vi "Host_main_Lab7.vi"() -> ()   [LabVIEW 2025]
uses:
  vi/thresholds.ctl
  RT_Cmd.ctl
  Command.ctl
  UI_Msg.ctl
  action.ctl
panel:
  out "error out":errorcluster
  in  "Manual trigger":bool
  in  "parameters":T1
  out "Waveform Graph":i16[][](graph)
  in  "Stop":bool
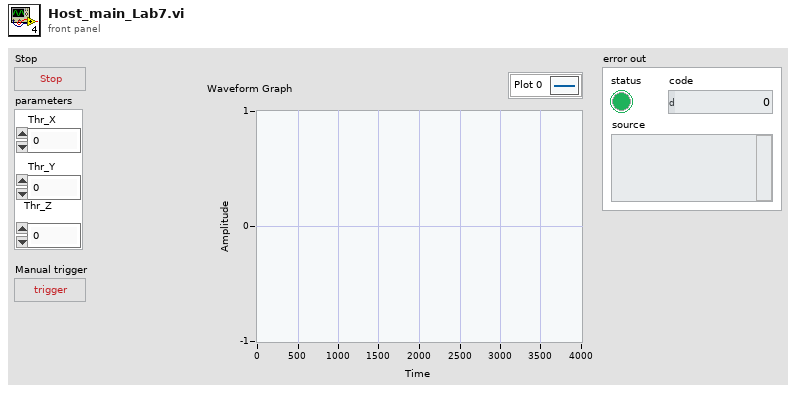
[diagram p1: front panel]
types:
  T1 = typedef "thresholds.ctl" = cluster{"Thr_X":i16, "Thr_Y":i16, "Thr_Z":i16}
  T2 = typedef "UI_Msg.ctl" = cluster{"action":T3, "Threshold":T1}
  T3 = typedef "action.ctl" = enum16{"Thresholds_Changed", "Manual_Trigger", "Stop"}
  T4 = typedef "RT_Cmd.ctl" = cluster{"command":T5, "parameters":T1}
  T5 = typedef "Command.ctl" = enum16{"threshold_config", "manual_trigger", "stop"}
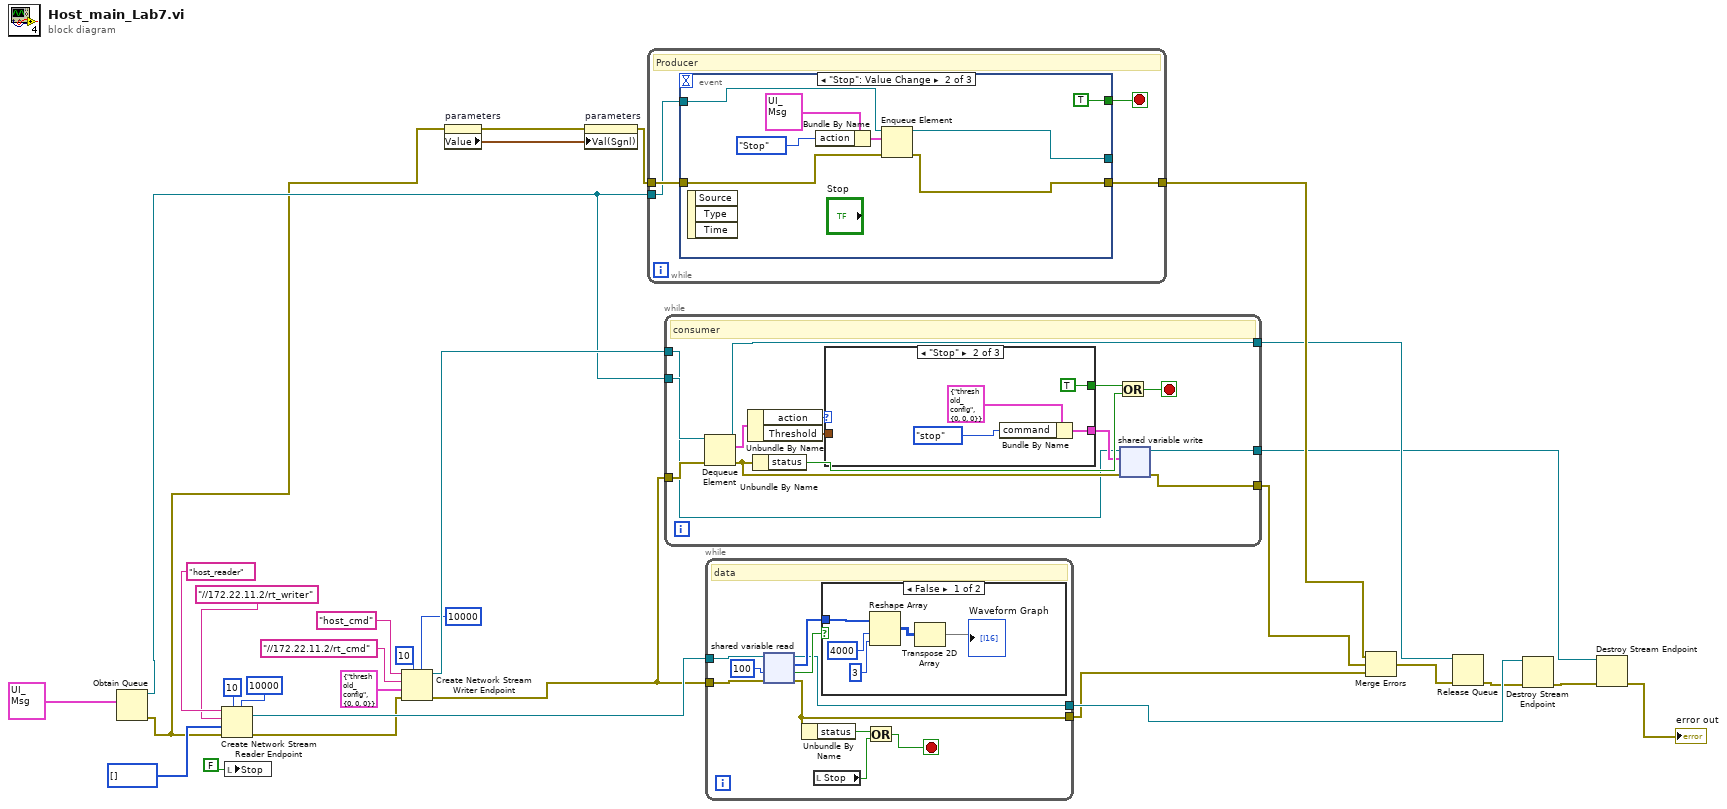
[diagram p0: block diagram]
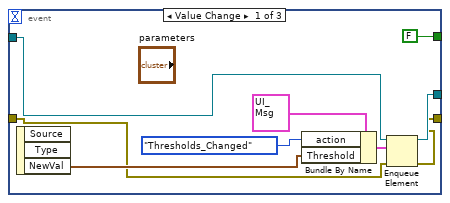
[diagram p2: hidden frame]
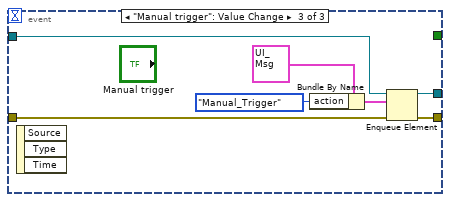
[diagram p3: hidden frame]
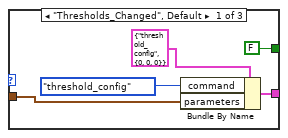
[diagram p4: hidden frame]
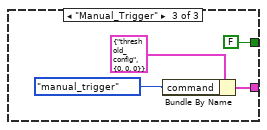
[diagram p5: hidden frame]
diagram:
  n1 = Obtain Queue(element data type=T2 {"action"=enum."Thresholds_Changed", "Threshold"={"Thr_X"=0, "Thr_Y"=0, "Thr_Z"=0}} ("msg")) -> (queue out=w5:refnum<queue>, error out=w2:errorcluster)  [unwired: 4 in, 1 out]
  n2 = Create Network Stream Reader Endpoint(5:10000 ("timeout in ms (-1)"), 7:10 ("reader buffer size"), 8:w2, 9:i16[] [], 10:"//172.22.11.2/rt_writer" ("writer url"), 11:"host_reader" ("writer name")) -> (0:w11:errorcluster, 3:w27:refnum<k21>)  [unwired: 1 in]
  n3 = local write "Stop"(FALSE ("Stop")) -> ()
  n4 = Create Network Stream Writer Endpoint(5:10000 ("timeout in ms (-1)"), 7:10 ("writer buffer size"), 8:w11, 9:T4 {"command"=enum."threshold_config", "parameters"={"Thr_X"=0, "Thr_Y"=0, "Thr_Z"=0}} ("data"), 10:"//172.22.11.2/rt_cmd" ("writer url"), 11:"host_cmd" ("writer name")) -> (0:w9:errorcluster, 3:w20:refnum<k21>)  [unwired: 1 in]
  n5 = property on="parameters" class="Clust (strict)"(error in=w2) -> (error out=w4:errorcluster, "Value"=w3:T1)  [unwired: 1 in, 1 out]
  n6 = property on="parameters" class="Clust (strict)"(error in=w4, "Val(Sgnl)"=w3) -> (error out=w1:errorcluster)  [unwired: 1 in, 1 out]
  n7 = while {
    tunnel: w1 -> [w34]
    tunnel: w5 -> [w32]
    tunnel: [w33] -> w17
    stop <- w35 stop-if-true
    # "Producer"
    n8 = event shown="[1] \"Stop\": Value Change" {
      selector: _ -> [_ _ _]
      dyn-events: _ -> [_ _ _]
      timeout: _ -> [_ _ _]
      tunnel: [FALSE TRUE _] -> w35
      tunnel: [w39 w48 w57] -> _
      tunnel: w34 -> [w38 w47 w56]
      tunnel: [w37 w46 w55] -> w33
      tunnel: w32 -> [w40 w49 w54]
      event Value Change {
        n9 = event-data() -> ("NewVal"=w41:T1)  [unwired: 1 in, 2 out]
        n10 = Bundle By Name(cluster=T2 {"action"=enum."Thresholds_Changed", "Threshold"={"Thr_X"=0, "Thr_Y"=0, "Thr_Z"=0}} ("msg"), "action"=action."Thresholds_Changed", "Threshold"=w41) -> (w43:T2)
        n11 = Enqueue Element(queue=w40, element=w43, error in (no error)=w38) -> (queue out=w39:refnum<queue>, error out=w37:errorcluster)  [unwired: 1 in, 1 out]
      }
      event "Stop": Value Change {
        n12 = event-data() -> ()  [unwired: 1 in, 3 out]
        n13 = Bundle By Name(cluster=T2 {"action"=enum."Thresholds_Changed", "Threshold"={"Thr_X"=0, "Thr_Y"=0, "Thr_Z"=0}} ("msg"), "action"=action."Stop") -> (w50:T2)
        n14 = Enqueue Element(queue=w49, element=w50, error in (no error)=w47) -> (queue out=w48:refnum<queue>, error out=w46:errorcluster)  [unwired: 1 in, 1 out]
      }
      event "Manual trigger": Value Change {
        n15 = event-data() -> ()  [unwired: 1 in, 3 out]
        n16 = Bundle By Name(cluster=T2 {"action"=enum."Thresholds_Changed", "Threshold"={"Thr_X"=0, "Thr_Y"=0, "Thr_Z"=0}} ("msg"), "action"=action."Manual_Trigger") -> (w59:T2)
        n17 = Enqueue Element(queue=w54, element=w59, error in (no error)=w56) -> (queue out=w57:refnum<queue>, error out=w55:errorcluster)  [unwired: 1 in, 1 out]
      }
    }
  }
  n18 = while {
    tunnel: w9 -> [w72]
    tunnel: w5 -> [w71]
    tunnel: [w63] -> w18
    tunnel: w20 -> [w62]
    tunnel: [w61] -> w15
    tunnel: [w60] -> w12
    stop <- w73 stop-if-true
    # "consumer"
    n19 = Dequeue Element(queue=w71, error in (no error)=w72) -> (queue out=w61:refnum<queue>, element=w70:T2, error out=w64:errorcluster)  [unwired: 1 in, 1 out]
    n20 = Unbundle By Name(w70) -> ("action"=w69:T3, "Threshold"=w66:T1)
    n21 = Unbundle By Name(w64) -> ("status"=w68:bool)
    n22 = case shown="\"Stop\"" w69 {
      tunnel: [FALSE TRUE FALSE] -> w67
      tunnel: [w75 w80 w84] -> w65
      tunnel: w66 -> [w76 _ _]
      frame "Thresholds_Changed", Default {
        n23 = Bundle By Name(cluster=T4 {"command"=enum."threshold_config", "parameters"={"Thr_X"=0, "Thr_Y"=0, "Thr_Z"=0}} ("data"), "command"=Command."threshold_config", "parameters"=w76) -> (w75:T4)
      }
      frame "Stop" {
        n24 = Bundle By Name(cluster=T4 {"command"=enum."threshold_config", "parameters"={"Thr_X"=0, "Thr_Y"=0, "Thr_Z"=0}} ("data"), "command"=Command."stop") -> (w80:T4)
      }
      frame "Manual_Trigger" {
        n25 = Bundle By Name(cluster=T4 {"command"=enum."threshold_config", "parameters"={"Thr_X"=0, "Thr_Y"=0, "Thr_Z"=0}} ("data"), "command"=Command."manual_trigger") -> (w84:T4)
      }
    }
    n26 = Or(x=w67, y=w68) -> (x .or. y?=w73:bool)
    n27 = shared-variable-write(w62, w64, w65) -> (w60:refnum<k21>, w63:errorcluster)  [unwired: 1 in, 1 out]
  }
  n28 = while {
    tunnel: w27 -> [w96]
    tunnel: w9 -> [w95]
    tunnel: [w91] -> w19
    tunnel: [w88] -> w26
    stop <- w92 stop-if-true
    # "data"
    n29 = shared-variable-read(w96, w95, 100 ("timeout ms (-1)")) -> (w88:refnum<k21>, w91:errorcluster, w90:bool, w89:i16[])
    n30 = Unbundle By Name(w91) -> ("status"=w93:bool)
    n31 = local read "Stop"() -> (w87:bool)
    n32 = case shown="False" w90 {
      tunnel: w89 -> [w101 _]
      frame False {
        n33 = Reshape Array(w101, 4000 ("dimension size"), 3 ("dimension size")) -> (w98:i16[][])
        n34 = Transpose 2D Array(2D array=w98) -> (transposed array=→"Waveform Graph":i16[][])
      }
      frame True {
      }
    }
    n35 = Or(x=w93, y=w87) -> (x .or. y?=w92:bool)
  }
  n36 = Merge Errors(w17, w18, w19) -> (w16:errorcluster)
  n37 = Release Queue(queue=w15, error in (no error)=w16) -> (error out=w14:errorcluster)  [unwired: 1 in, 2 out]
  n38 = Destroy Stream Endpoint(8:w14, 11:w26) -> (0:w13:errorcluster)
  n39 = Destroy Stream Endpoint(8:w13, 11:w12) -> (0:→"error out":errorcluster)
